vi "Load SA Precision Setting.vi"(8 "error in (no error)":errorcluster caption="에러 입력(에러 없음)", 9 "Sweep Time(sec)":dbl, 10 "Center Frequency":dbl, 11 "Instrument Manager 입력":refnum<class "Instrument Manager.lvclass">) -> (0 "error out":errorcluster caption="에러 출력", 3 "Instrument Manager 출력":refnum<class "Instrument Manager.lvclass">)   [LabVIEW 2023, in "Instrument Manager.lvclass"]
uses:
  Instrument Manager.lvclass
  Module/Spectrum Analyzer/TYPE DEFINITION/TYPE Detect Mode Select.ctl
  Module/Spectrum Analyzer/TYPE DEFINITION/TYPE Display Trace Mode Select.ctl
  042d5d38-4e5a-4ffb-96df-cc2328cc6af4.vi
  Instrument Manager.lvclass/Instrument Manager.ctl
  Module/Spectrum Analyzer/Spectrum Analyzer.lvlib
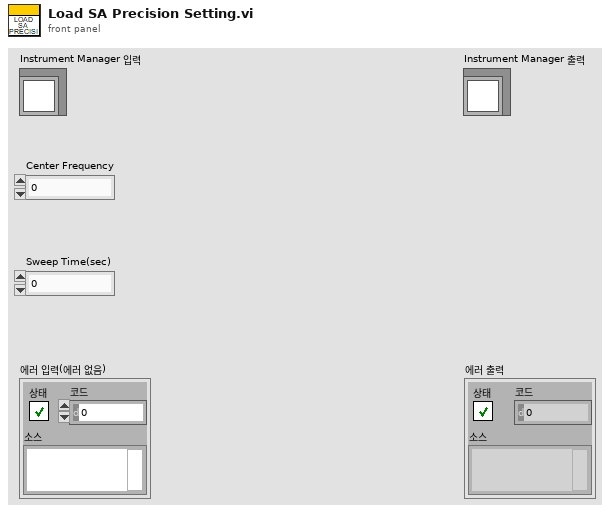
[diagram p1: front panel]
types:
  T1 = typedef "Spectrum Analyzer.lvlib/TYPE Display Trace Mode Select.ctl" = enum16{"Clear Write", "Max Hold", "Min Hold", "Average", "View"}
  T2 = typedef "Spectrum Analyzer.lvlib/TYPE Detect Mode Select.ctl" = enum16{"Det Auto (Normal)", "Auto Peak", "Positive Peak", "Negative Peak", "Sample", "RMS", "Average", "Quasipeak", "CISPR Average", "RMS Average"}
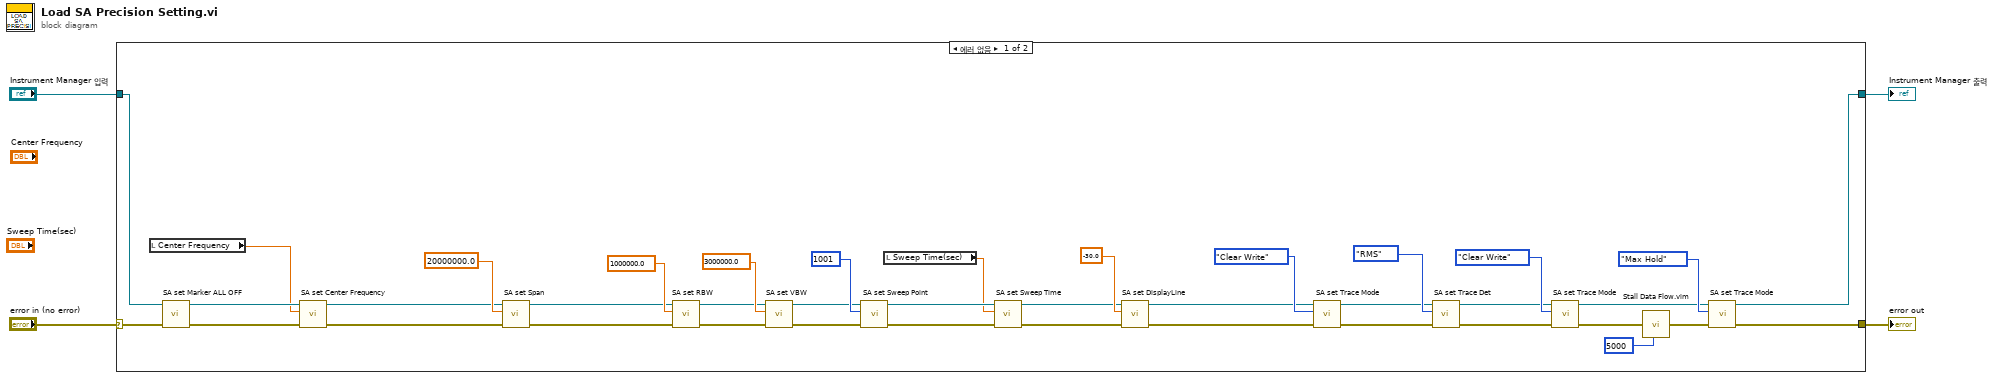
[diagram p0: block diagram]
diagram:
  n1 = case shown="에러 없음" "error in (no error)" {
    selector: "error in (no error)" -> [w43 w45]
    tunnel: [w21 w45] -> w3
    tunnel: [w9 w44] -> w1
    tunnel: "Instrument Manager 입력" -> [w19 w44]
    frame No Error {
      n2 = local read "Center Frequency"() -> (w7:dbl)
      n3 = call "SA set Marker ALL OFF.vi"("error in (no error)"=w43, "Instrument Manager 입력"=w19) -> ("error out"=w42:errorcluster, "Instrument Manager 출력"=w18:refnum<class "Instrument Manager.lvclass">)  [unwired: 8 in]
      n4 = call "SA set Center Frequency.vi"("error in (no error)"=w42, "Center Frequency (Hz)"=w7, "Instrument Manager 입력"=w18) -> ("error out"=w41:errorcluster, "Instrument Manager 출력"=w17:refnum<class "Instrument Manager.lvclass">)  [unwired: 7 in]
      n5 = call "SA set Span.vi"("error in (no error)"=w41, "Span (Hz)"=20000000.0 ("Center Frequency (Hz)"), "Instrument Manager 입력"=w17) -> ("error out"=w5:errorcluster, "Instrument Manager 출력"=w6:refnum<class "Instrument Manager.lvclass">)  [unwired: 7 in]
      n6 = call "SA set RBW.vi"("error in (no error)"=w5, "BW Value (Hz)"=1000000.0, "Instrument Manager 입력"=w6) -> ("error out"=w40:errorcluster, "Instrument Manager 출력"=w16:refnum<class "Instrument Manager.lvclass">)  [unwired: 7 in]
      n7 = call "SA set VBW.vi"("error in (no error)"=w40, "BW Value (Hz)"=3000000.0, "Instrument Manager 입력"=w16) -> ("error out"=w39:errorcluster, "Instrument Manager 출력"=w15:refnum<class "Instrument Manager.lvclass">)  [unwired: 7 in]
      n8 = call "SA set Sweep Point.vi"("error in (no error)"=w39, "Sweep Point"=u32 1001, "Instrument Manager 입력"=w15) -> ("error out"=w33:errorcluster, "Instrument Manager 출력"=w14:refnum<class "Instrument Manager.lvclass">)  [unwired: 7 in]
      n9 = local read "Sweep Time(sec)"() -> (w8:dbl)
      n10 = call "SA set Sweep Time.vi"("error in (no error)"=w33, "Sweep Time(sec)"=w8, "Instrument Manager 입력"=w14) -> ("error out"=w32:errorcluster, "Instrument Manager 출력"=w13:refnum<class "Instrument Manager.lvclass">)  [unwired: 7 in]
      n11 = call "SA set DisplayLine.vi"("error in (no error)"=w32, "Amplitude"=-30.0, "Instrument Manager 입력"=w13) -> ("error out"=w30:errorcluster, "Instrument Manager 출력"=w27:refnum<class "Instrument Manager.lvclass">)  [unwired: 7 in]
      n12 = call "SA set Trace Mode.vi"("error in (no error)"=w30, "Trace Mode"=TYPE_Display_Trace_Mode_Select."Clear Write", "Instrument Manager 입력"=w27) -> ("error out"=w26:errorcluster, "Instrument Manager 출력"=w12:refnum<class "Instrument Manager.lvclass">)  [unwired: 7 in]
      n13 = call "SA set Trace Det.vi"("error in (no error)"=w26, "Detector Type"=TYPE_Detect_Mode_Select."RMS", "Instrument Manager 입력"=w12) -> ("error out"=w25:errorcluster, "Instrument Manager 출력"=w11:refnum<class "Instrument Manager.lvclass">)  [unwired: 7 in]
      n14 = call "SA set Trace Mode.vi"("error in (no error)"=w25, "Trace Mode"=TYPE_Display_Trace_Mode_Select."Clear Write", "Instrument Manager 입력"=w11) -> ("error out"=w23:errorcluster, "Instrument Manager 출력"=w10:refnum<class "Instrument Manager.lvclass">)  [unwired: 7 in]
      n15 = call "Stall Data Flow.vim"("value in"=w23, "milliseconds to wait"=u32 5000) -> ("value out"=w22:errorcluster)  [unwired: 1 out]
      n16 = call "SA set Trace Mode.vi"("error in (no error)"=w22, "Trace Mode"=TYPE_Display_Trace_Mode_Select."Max Hold", "Instrument Manager 입력"=w10) -> ("error out"=w21:errorcluster, "Instrument Manager 출력"=w9:refnum<class "Instrument Manager.lvclass">)  [unwired: 7 in]
    }
    frame Error {
    }
  }
  "error out" <- w3
  "Instrument Manager 출력" <- w1
